vi "analyze memory usage.vi"(8 "error in (no error)":errorcluster, 10 "offset (0)":i64, 11 "file path":path) -> (0 "error out":errorcluster, 2 "memory stats":T1, 3 "Data":dbl[](array[numeric]))   [LabVIEW 2014]
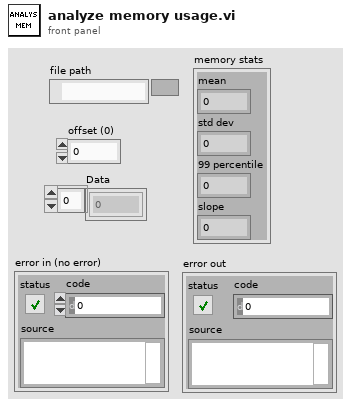
[diagram p1: front panel]
types:
  T1 = cluster{"mean":dbl, "std dev":dbl, "99 percentile":dbl, "slope":dbl}
  T2 = cluster{"mean":dbl, "std dev":dbl, "99th percentile":dbl, "slope":dbl}
  T3 = cluster{"mean":dbl, "standard deviation":dbl, "calculated percentiles":dbl[], "slope":dbl, "max":dbl}
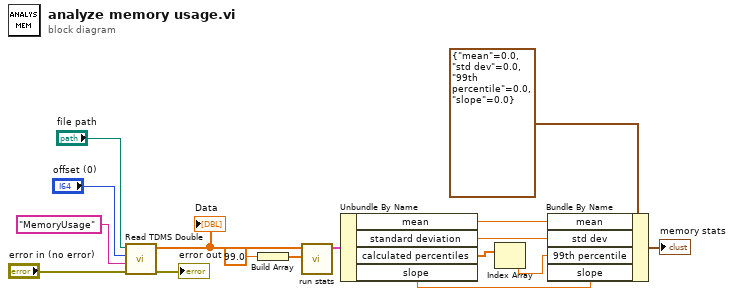
[diagram p0: block diagram]
diagram:
  n1 = call "Read TDMS Double.vi"("error in (no error)"="error in (no error)", "channel name(s) in"="MemoryUsage", "offset (0)"="offset (0)", "file path"="file path") -> ("error out"=→"error out":errorcluster, "Data"=w7:dbl[])  [unwired: 6 in]
  "Data" <- w7
  n2 = Build Array(99.0 ("p")) -> (w8:dbl[])
  n3 = call "run stats.vi"("percentiles"=w8, "Data"=w7) -> ("stats out"=w6:T3)  [unwired: 9 in]
  n4 = Unbundle By Name(w6) -> ("mean"=w4:dbl, "standard deviation"=w3:dbl, "calculated percentiles"=w5:dbl[], "slope"=w1:dbl)
  n5 = Index Array(array=w5) -> (element=w2:dbl)  [unwired: 1 in]
  n6 = Bundle By Name(cluster=T2 {"mean"=0.0, "std dev"=0.0, "99th percentile"=0.0, "slope"=0.0}, "mean"=w4, "std dev"=w3, "99th percentile"=w2, "slope"=w1) -> (→"memory stats":T2)
